vi "Read XNET Session.vi"(8 "error in (no error)":errorcluster, 11 "XNET_CAN_RW in":refnum<class "XNET CAN RW.lvclass">) -> (0 "error out":errorcluster, 2 "XNET Session":refnum<k21>, 3 "XNET_CAN_RW out":refnum<class "XNET CAN RW.lvclass">)   [LabVIEW 2021, in "XNET CAN RW.lvclass"]
uses:
  XNET CAN RW.lvclass
  XNET CAN RW.lvclass/XNET CAN RW.ctl
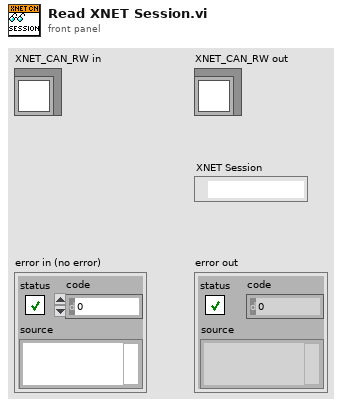
[diagram p1: front panel]
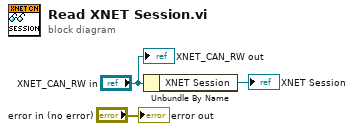
[diagram p0: block diagram]
diagram:
  n1 = Unbundle By Name("XNET_CAN_RW in") -> ("XNET Session"=→"XNET Session":refnum<k21>)
  "error out" <- "error in (no error)"
  "XNET_CAN_RW out" <- "XNET_CAN_RW in"
